vi "Combine_Anomaly_Detection_Results.vi"(4 "Relative Resolution":sgl=1.0, 5 "Evaluation_Results":T8 {"Pixel_Range"."Min" format="%#_5g"}, 6 "Display_Options":T1={"ROI_Options"={"Color"=16711680, "Width"=3, "Drawing Mode"=enum."Frame"}, "Heatmap_Options"={"ColorMap"=enum."Jet", "Alpha"=0.4, "Heatmap Range"={"Min"=-1.0, "Max"=-1.0}}, "Report_Images_CFG"={"Original Image"=TRUE, "Ground Truth"=FALSE, "HeatMap"=TRUE, "Mask"=FALSE, "Segmentation"=TRUE}} {"Heatmap_Options"."Heatmap Range"."Min" format="%#_5g"}, 7 "Pixel Anomaly Thrshld":sgl=-1.0 format="%_4g", 8 "error in":errorcluster, 9 "Anomaly Map":sgl[][](array[numeric])=array320x272[87040 elements], 10 "Gt File Path":path=path "D:/DNN/AD/Ngene/Cards_3OfSpades/01_Vertical_Filtered/Test/good/good_2069.bmp", 11 "Orig Image In":T7=refnum) -> (0 "error out":errorcluster, 2 "Actual Pixel Threshold":sgl=7.2, 3 "Anomaly Detection Results":T9={"Image"="remote image 00000241F53A1FE8", "Ground Truth"=refnum, "Predicted Heat Map"="remote image 00000241C7A9E038", "Predicted Mask"=refnum, "Segmentation"="remote image 00000241F8ADE158"})   [LabVIEW 2020]
uses:
  Controls/Anomaly_Detection_Results_Imgs.ctl
  <vilib>/Ngene/DeepLTK Anomaly Detection Addon/Toolkit/API/Controls/NNPC_Evaluation_Results.ctl
  <vilib>/vision/Image Controls.llb/IMAQ Image.ctl
  Controls/Display_Options.ctl
  Controls/ROI_Display_Options.ctl
  Controls/Heatmap_Display_Options.ctl
  Controls/ColorMap.ctl
  <vilib>/Ngene/DeepLTK Anomaly Detection Addon/Toolkit/API/Controls/MinMax.ctl
  Controls/Report_Images_CFG.ctl
  <vilib>/vision/NI_Vision_Development_Module.lvlib
  <vilib>/Ngene/DeepLTK Anomaly Detection Addon/Toolkit/DeepLTK_Anomaly_Detection_Addon.lvlib
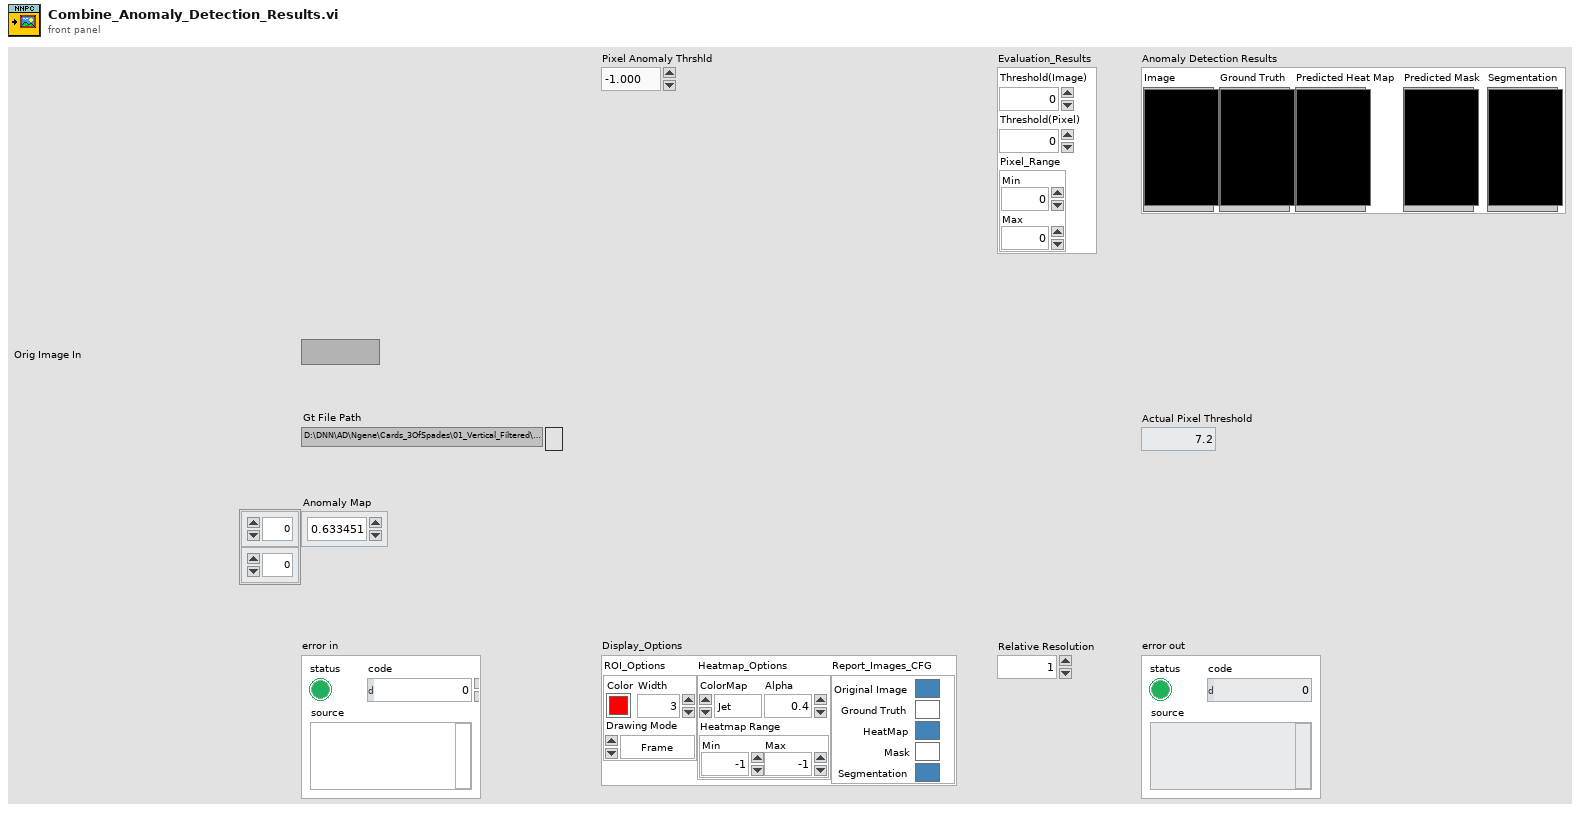
[diagram p1: front panel]
types:
  T1 = typedef "Display_Options.ctl" = cluster{"ROI_Options":T2, "Heatmap_Options":T3, "Report_Images_CFG":T6}
  T2 = typedef "ROI_Display_Options.ctl" = cluster{"Color":u32, "Width":u32, "Drawing Mode":enum16{"Frame", "Fill"}}
  T3 = typedef "Heatmap_Display_Options.ctl" = cluster{"ColorMap":T4, "Alpha":sgl, "Heatmap Range":T5}
  T4 = typedef "ColorMap.ctl" = enum16{"Jet", "Perula", "Inferno", "Plasma", "Viridis"}
  T5 = typedef "DeepLTK_Anomaly_Detection_Addon.lvlib/MinMax.ctl" = cluster{"Min":sgl, "Max":sgl}
  T6 = typedef "Report_Images_CFG.ctl" = cluster{"Original Image":bool, "Ground Truth":bool, "HeatMap":bool, "Mask":bool, "Segmentation":bool}
  T7 = typedef "IMAQ Image.ctl" = refnum<image>
  T8 = typedef "DeepLTK_Anomaly_Detection_Addon.lvlib/NNPC_Evaluation_Results.ctl" = cluster{"Threshold(Image)":sgl, "Threshold(Pixel)":sgl, "Pixel_Range":cluster{"Min":sgl, "Max":sgl}}
  T9 = typedef "Anomaly_Detection_Results_Imgs.ctl" = cluster{"Image":T7, "Ground Truth":T7, "Predicted Heat Map":T7, "Predicted Mask":T7, "Segmentation":T7}
  T10 = typedef "Image Type" = u32
  T11 = typedef "ROI Descriptor" = cluster{"Global Rectangle":i32[], "Contours":cluster{"ID":enum32{"External", "Internal"}, "Type":u32, "Coordinates":i32[]}[]}
  T12 = cluster{"ID":enum32{"External", "Internal"}, "Type":u32, "Coordinates":i32[]}[]
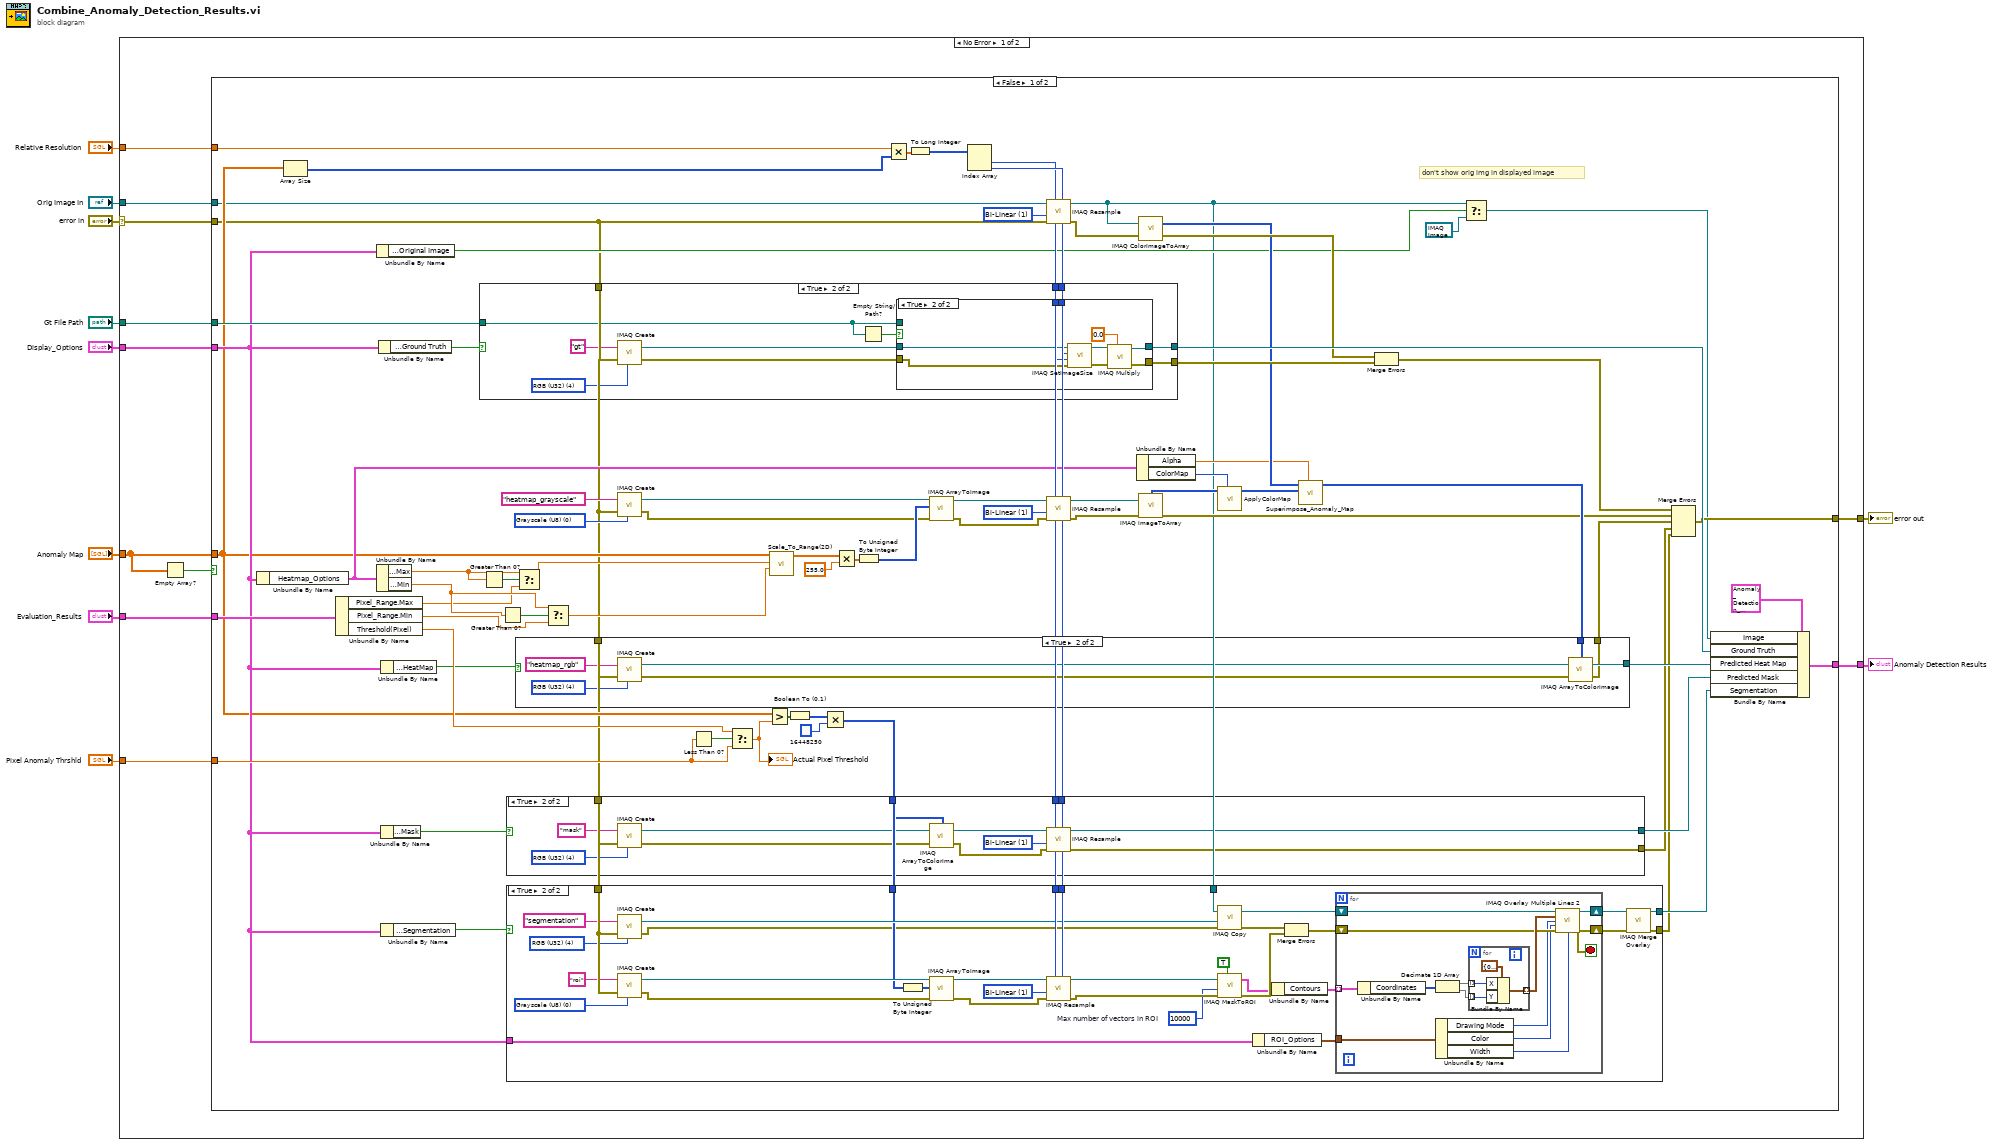
[diagram p0: block diagram]
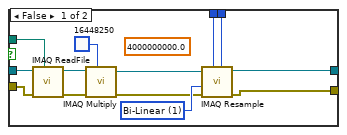
[diagram p6: hidden frame]
diagram:
  n1 = case shown="No Error" "error in" {
    selector: "error in" -> [w13 w203]
    tunnel: [w21 _] -> w10
    tunnel: "Display_Options" -> [w12 _]
    tunnel: "Pixel Anomaly Thrshld" -> [w20 _]
    tunnel: "Gt File Path" -> [w19 _]
    tunnel: [w16 w203] -> w6
    tunnel: "Anomaly Map" -> [w15 _]
    tunnel: "Evaluation_Results" -> [w18 _]
    tunnel: "Relative Resolution" -> [w17 _]
    tunnel: "Orig Image In" -> [w14 _]
    frame No Error {
      n2 = Empty Array?(array=w15) -> (empty?=w11:bool)
      n3 = case shown="False" w11 {
        tunnel: [w92 _] -> w21
        tunnel: w20 -> [w88 _]
        tunnel: w19 -> [w84 _]
        tunnel: w18 -> [w83 _]
        tunnel: w17 -> [w82 _]
        tunnel: [w76 w202] -> w16
        tunnel: w15 -> [w26 _]
        tunnel: w14 -> [w23 _]
        tunnel: w13 -> [w24 w202]
        tunnel: w12 -> [w71 _]
        frame False {
          w53 = u32 1 items=["Zero Order", "Bi-Linear", "Quadratic", "Cubic Spline"] ("Interpolation Type")
          w57 = T10 0 items=["Grayscale (U8)", "Grayscale (I16)", "Grayscale (SGL)", "Complex (CSG)", "RGB (U32)", "HSL (U32)", "RGB (U64)", "Grayscale (U16)"] ("Image Type")
          w86 = u32 1 items=["Zero Order", "Bi-Linear", "Quadratic", "Cubic Spline"] ("Interpolation Type")
          # "don't show orig img in displayed image"
          n4 = Unbundle By Name(w71) -> ("Heatmap_Options"=w31:T3)
          n5 = Array Size(array=w26) -> (size(s)=w25:i32[])
          n6 = Unbundle By Name(w83) -> ("Pixel_Range.Max"=w36:sgl, "Pixel_Range.Min"=w35:sgl, "Threshold(Pixel)"=w34:sgl)
          n7 = Unbundle By Name(w71) -> ("Report_Images_CFG.Original Image"=w69:bool)
          n8 = Unbundle By Name(w31) -> ("Heatmap Range.Max"=w37:sgl, "Heatmap Range.Min"=w38:sgl)
          n9 = Unbundle By Name(w71) -> ("Report_Images_CFG.Ground Truth"=w75:bool)
          n10 = Unbundle By Name(w71) -> ("Report_Images_CFG.HeatMap"=w27:bool)
          n11 = Unbundle By Name(w71) -> ("Report_Images_CFG.Mask"=w28:bool)
          n12 = Unbundle By Name(w71) -> ("Report_Images_CFG.Segmentation"=w30:bool)
          n13 = Greater Than 0?(x=w37) -> (x > 0?=w41:bool)
          n14 = Greater Than 0?(x=w38) -> (x > 0?=w39:bool)
          n15 = Select(t=w37, s=w41, f=w36) -> (s? t:f=w42:sgl)
          n16 = Select(t=w38, s=w39, f=w35) -> (s? t:f=w40:sgl)
          n17 = call "IMAQ Create"("Image Name"="heatmap_grayscale", "Image Type"=w57, "error in (no error)"=w24) -> ("New Image"=w56:T7, "error out"=w47:errorcluster)  [unwired: 2 in]
          n18 = Less Than 0?(x=w88) -> (x < 0?=w50:bool)
          n19 = Select(t=w34, s=w50, f=w88) -> (s? t:f=w49:sgl)
          "Actual Pixel Threshold" <- w49
          n20 = Greater?(x=w26, y=w49) -> (0:w64:bool[][])
          n21 = call "Scale_To_Range(2D).vi"("min pixel score"=w40, "max pixel score"=w42, "anomaly map"=w26) -> ("anomaly map normalized"=w67:sgl[][])  [unwired: 8 in]
          n22 = Boolean To (0,1)(Boolean=w64) -> (0, 1=w65:i16[][])
          n23 = Multiply(x=w65, y=u32 16448250) -> (x*y=w29:u32[][])
          n24 = Multiply(x=w67, y=sgl 255.0) -> (x*y=w60:sgl[][])
          n25 = To Unsigned Byte Integer(number=w60) -> (unsigned 8bit integer=w59:u8[][])
          n26 = Multiply(x=w82, y=w25) -> (x*y=w79:sgl[])
          n27 = To Long Integer(number=w79) -> (32bit integer=w78:i32[])
          n28 = call "IMAQ ArrayToImage"("error in (no error)"=w47, "Image Pixels (U8)"=w59, "Image"=w56) -> ("error out"=w48:errorcluster, "Image Out"=w55:T7)  [unwired: 7 in]
          n29 = Index Array(array=w78) -> (element #1=w80:i32, element #2=w81:i32)  [unwired: 2 in]
          n30 = case shown="True" w75 {
            tunnel: [_ w177] -> w87
            tunnel: w24 -> [w168 w174]
            tunnel: w84 -> [_ w173]
            tunnel: w81 -> [_ w171]
            tunnel: w80 -> [_ w170]
            tunnel: [w168 w169] -> w77
            frame False {
              # "don't show GT in displayed image"
            }
            frame True {
              w178 = T10 4 items=["Grayscale (U8)", "Grayscale (I16)", "Grayscale (SGL)", "Complex (CSG)", "RGB (U32)", "HSL (U32)", "RGB (U64)", "Grayscale (U16)"] ("Image Type")
              n31 = call "IMAQ Create"("Image Name"="gt", "Image Type"=w178, "error in (no error)"=w174) -> ("New Image"=w175:T7, "error out"=w172:errorcluster)  [unwired: 2 in]
              n32 = Empty String/Path?(string/path=w173) -> (empty?=w176:bool)
              n33 = case shown="True" w176 {
                tunnel: w175 -> [w192 w201]
                tunnel: w173 -> [w191 _]
                tunnel: [w190 w195] -> w177
                tunnel: [w189 w194] -> w169
                tunnel: w171 -> [w188 w200]
                tunnel: w170 -> [w187 w199]
                tunnel: w172 -> [w185 w193]
                frame False {
                  (unwired) 4000000000.0 ("Constant")
                  w186 = u32 1 items=["Zero Order", "Bi-Linear", "Quadratic", "Cubic Spline"] ("Interpolation Type")
                  n34 = call "IMAQ ReadFile"("File Path"=w191, "error in (no error)"=w185, "Image"=w192) -> ("error out"=w183:errorcluster, "Image Out"=w184:T7)  [unwired: 4 in, 3 out]
                  n35 = call "IMAQ Multiply"("Image Src A"=w184, "Constant"=u32 16448250, "error in (no error)"=w183) -> ("Image Dst Out"=w181:T7, "error out"=w182:errorcluster)  [unwired: 4 in]
                  n36 = call "IMAQ Resample"("X Resolution"=w188, "Y Resolution"=w187, "error in (no error)"=w182, "Interpolation Type"=w186, "Image Src"=w181) -> ("error out"=w189:errorcluster, "Image Dst Out"=w190:T7)  [unwired: 5 in]
                }
                frame True {
                  n37 = call "IMAQ SetImageSize"("error in (no error)"=w193, "Y Resolution"=w199, "X Resolution"=w200, "Image"=w201) -> ("error out"=w198:errorcluster, "Image Out"=w197:T7)  [unwired: 1 in]
                  n38 = call "IMAQ Multiply"("Image Src A"=w197, "Constant"=0.0, "error in (no error)"=w198) -> ("Image Dst Out"=w195:T7, "error out"=w194:errorcluster)  [unwired: 4 in]
                }
              }
            }
          }
          n39 = case shown="True" w28 {
            tunnel: [_ w116] -> w89
            tunnel: w24 -> [w103 w115]
            tunnel: w81 -> [_ w114]
            tunnel: w80 -> [_ w113]
            tunnel: [w103 w105] -> w45
            tunnel: w29 -> [_ w104]
            frame False {
              # "don't show Mask in displayed image"
            }
            frame True {
              w109 = u32 1 items=["Zero Order", "Bi-Linear", "Quadratic", "Cubic Spline"] ("Interpolation Type")
              w112 = T10 4 items=["Grayscale (U8)", "Grayscale (I16)", "Grayscale (SGL)", "Complex (CSG)", "RGB (U32)", "HSL (U32)", "RGB (U64)", "Grayscale (U16)"] ("Image Type")
              n40 = call "IMAQ Create"("Image Name"="mask", "Image Type"=w112, "error in (no error)"=w115) -> ("New Image"=w110:T7, "error out"=w107:errorcluster)  [unwired: 2 in]
              n41 = call "IMAQ ArrayToColorImage"("Image Pixels (U32)"=w104, "Image"=w110, "error in (no error)"=w107) -> ("Image Out"=w108:T7, "error out"=w106:errorcluster)  [unwired: 2 in]
              n42 = call "IMAQ Resample"("X Resolution"=w114, "Y Resolution"=w113, "error in (no error)"=w106, "Interpolation Type"=w109, "Image Src"=w108) -> ("error out"=w105:errorcluster, "Image Dst Out"=w116:T7)  [unwired: 5 in]
            }
          }
          n43 = call "IMAQ Resample"("X Resolution"=w81, "Y Resolution"=w80, "error in (no error)"=w24, "Interpolation Type"=w86, "Image Src"=w23) -> ("error out"=w85:errorcluster, "Image Dst Out"=w22:T7)  [unwired: 5 in]
          n44 = case shown="True" w30 {
            tunnel: [_ w150] -> w91
            tunnel: w22 -> [_ w149]
            tunnel: w24 -> [w117 w148]
            tunnel: w81 -> [_ w147]
            tunnel: w80 -> [_ w146]
            tunnel: w29 -> [_ w138]
            tunnel: [w117 w128] -> w46
            tunnel: w71 -> [_ w119]
            frame False {
              # "don't show Segmentation in displayed image"
            }
            frame True {
              w118 = 10000  # Max number of vectors in ROI
              w132 = u32 1 items=["Zero Order", "Bi-Linear", "Quadratic", "Cubic Spline"] ("Interpolation Type")
              w141 = T10 4 items=["Grayscale (U8)", "Grayscale (I16)", "Grayscale (SGL)", "Complex (CSG)", "RGB (U32)", "HSL (U32)", "RGB (U64)", "Grayscale (U16)"] ("Image Type")
              w144 = T10 0 items=["Grayscale (U8)", "Grayscale (I16)", "Grayscale (SGL)", "Complex (CSG)", "RGB (U32)", "HSL (U32)", "RGB (U64)", "Grayscale (U16)"] ("Image Type")
              n45 = call "IMAQ Create"("Image Name"="segmentation", "Image Type"=w141, "error in (no error)"=w148) -> ("New Image"=w139:T7, "error out"=w129:errorcluster)  [unwired: 2 in]
              n46 = call "IMAQ Create"("Image Name"="roi", "Image Type"=w144, "error in (no error)"=w148) -> ("New Image"=w143:T7, "error out"=w130:errorcluster)  [unwired: 2 in]
              n47 = To Unsigned Byte Integer(number=w138) -> (unsigned 8bit integer=w137:u8[][])
              n48 = call "IMAQ ArrayToImage"("error in (no error)"=w130, "Image Pixels (U8)"=w137, "Image"=w143) -> ("error out"=w131:errorcluster, "Image Out"=w135:T7)  [unwired: 7 in]
              n49 = call "IMAQ Resample"("X Resolution"=w147, "Y Resolution"=w146, "error in (no error)"=w131, "Interpolation Type"=w132, "Image Src"=w135) -> ("error out"=w134:errorcluster, "Image Dst Out"=w136:T7)  [unwired: 5 in]
              n50 = call "IMAQ Copy"("error in (no error)"=w129, "Image Dst"=w139, "Image Src"=w149) -> ("error out"=w127:errorcluster, "Image Dst Out"=w124:T7)  [unwired: 3 in]
              n51 = call "IMAQ MaskToROI"("External edges only (T)"=TRUE, "Image"=w136, "Max number of vectors in ROI"=w118, "error in (no error)"=w134) -> ("ROI Descriptor"=w126:T11, "error out"=w133:errorcluster)  [unwired: 3 in, 1 out]
              n52 = Unbundle By Name(w119) -> ("ROI_Options"=w120:T2)
              n53 = Unbundle By Name(w126) -> ("Contours"=w125:T12)
              n54 = Merge Errors(w127, w133) -> (w122:errorcluster)
              n55 = for {
                tunnel: w125 -> [w163] mode=indexing
                shift-right: [w151] -> w121
                shift-left: w122 -> [w156]
                tunnel: w120 -> [w155]
                shift-right: [w157] -> w123
                shift-left: w124 -> [w158]
                stop <- w151 stop-if-true
                n56 = Unbundle By Name(w163) -> ("Coordinates"=w162:i32[])
                n57 = Decimate 1D Array(w162) -> (w161:i32[], w160:i32[])
                n58 = Unbundle By Name(w155) -> ("Drawing Mode"=w154:enum16{"Frame", "Fill"}, "Color"=w153:u32, "Width"=w152:u32)
                n59 = for {
                  tunnel: w161 -> [w166] mode=indexing
                  tunnel: w160 -> [w165] mode=indexing
                  tunnel: [w164] -> w159 mode=indexing
                  n60 = Bundle By Name(cluster=cluster{"X":dbl, "Y":dbl} {"X"=0.0, "Y"=0.0} ("Line End Points"), "X"=w166, "Y"=w165) -> (w164:cluster{"X":dbl, "Y":dbl})
                }
                n61 = call "IMAQ Overlay Multiple Lines 2"("Image"=w158, "Line End Points"=w159, "Drawing Mode (Frame)"=w154, "Color"=w153, "error in (no error)"=w156, "Width"=w152) -> ("Image Out"=w157:T7, "error out"=w151:errorcluster)  [unwired: 8 in]
              }
              n62 = call "IMAQ Merge Overlay"("error in (no error)"=w121, "Image Src"=w123) -> ("error out"=w128:errorcluster, "Image Dst Out"=w150:T7)  [unwired: 8 in]
            }
          }
          n63 = call "IMAQ Resample"("X Resolution"=w81, "Y Resolution"=w80, "error in (no error)"=w48, "Interpolation Type"=w53, "Image Src"=w55) -> ("error out"=w52:errorcluster, "Image Dst Out"=w54:T7)  [unwired: 5 in]
          n64 = Unbundle By Name(w31) -> ("Alpha"=w33:sgl, "ColorMap"=w32:T4)
          n65 = call "IMAQ ColorImageToArray"("Image"=w22, "error in (no error)"=w85) -> ("Image Pixels (U32)"=w72:u32[][], "error out"=w73:errorcluster)  [unwired: 2 in, 1 out]
          n66 = call "IMAQ ImageToArray"("error in (no error)"=w52, "Image"=w54) -> ("error out"=w43:errorcluster, "Image Pixels (U8)"=w51:u8[][])  [unwired: 2 in, 3 out]
          n67 = call "ApplyColorMap.vi"("ColorMap Type"=w32, "Image in"=w51) -> ("Image out"=w62:u32[][])  [unwired: 9 in]
          n68 = call "Superimpose_Anomaly_Map.vi"("Alpha"=w33, "Anomaly Map"=w62, "Image"=w72) -> ("Img out"=w63:u32[][])  [unwired: 8 in]
          n69 = case shown="True" w27 {
            tunnel: [_ w102] -> w90
            tunnel: w24 -> [w94 w101]
            tunnel: w63 -> [_ w100]
            tunnel: [w94 w95] -> w44
            frame False {
              # "don't show HeatMap in displayed image"
            }
            frame True {
              w98 = T10 4 items=["Grayscale (U8)", "Grayscale (I16)", "Grayscale (SGL)", "Complex (CSG)", "RGB (U32)", "HSL (U32)", "RGB (U64)", "Grayscale (U16)"] ("Image Type")
              n70 = call "IMAQ Create"("Image Name"="heatmap_rgb", "Image Type"=w98, "error in (no error)"=w101) -> ("New Image"=w97:T7, "error out"=w96:errorcluster)  [unwired: 2 in]
              n71 = call "IMAQ ArrayToColorImage"("Image Pixels (U32)"=w100, "Image"=w97, "error in (no error)"=w96) -> ("Image Out"=w102:T7, "error out"=w95:errorcluster)  [unwired: 2 in]
            }
          }
          n72 = Merge Errors(w73, w77) -> (w74:errorcluster)
          n73 = Select(t=w22, s=w69, f=T7 refnum ("Image Dst Out")) -> (s? t:f=w70:T7)
          n74 = Merge Errors(w74, w43, w44, w45, w46) -> (w76:errorcluster)
          n75 = Bundle By Name(cluster=T9 {"Image"=refnum, "Ground Truth"=refnum, "Predicted Heat Map"=refnum, "Predicted Mask"=refnum, "Segmentation"=refnum} ("Anomaly Detection Results"), "Image"=w70, "Ground Truth"=w87, "Predicted Heat Map"=w90, "Predicted Mask"=w89, "Segmentation"=w91) -> (w92:T9)
        }
        frame True {
        }
      }
    }
    frame Error {
    }
  }
  "error out" <- w6
  "Anomaly Detection Results" <- w10
